vi "RemoteVI Window Rows.vi"(0 "raw":T2(array[cluster]), 1 "labview only?":bool, 2 "skip":u64) -> (4 "rows":T1(array[cluster]))   [LabVIEW 2020, in "RemoteVI.lvlib"]
doc: "The windows RemoteVI Server offers to share, grouped and sorted, from the top-level windows RemoteVI List Top Windows.vi read. Kept: visible, at least 100 x 50 pixels, with a caption, not a tool window (WS_EX_TOOLWINDOW) nor one that cannot be activated (WS_EX_NOACTIVATE), not a shell window (classes Windows.UI.Core.CoreWindow, Windows.Internal.Shell.TabProxyWindow, Progman, LockScreenBackstopFrame); a LabVIEW window (class LVDChild) also when it is owned (LabVIEW's panels are owned by its hidden frame window), other windows only when they are not owned (no dialogs); no LabVIEW window whose caption names a Block Diagram or Project Explorer; not the window skip (the app's own). group 0 = LabVIEW (the development environment, LabVIEW.exe), 1 = a LabVIEW-built application (a LabVIEW window of another program), 2 = other programs; labview only? keeps groups 0 and 1. Sorted by group, program name (case-insensitive) and caption. Pure function, cannot fail. Reference: windowRows() in tools\\lib\\server-app.mjs, vectors tests\\vectors\\server-app.json."
uses:
  RemoteVI.lvlib
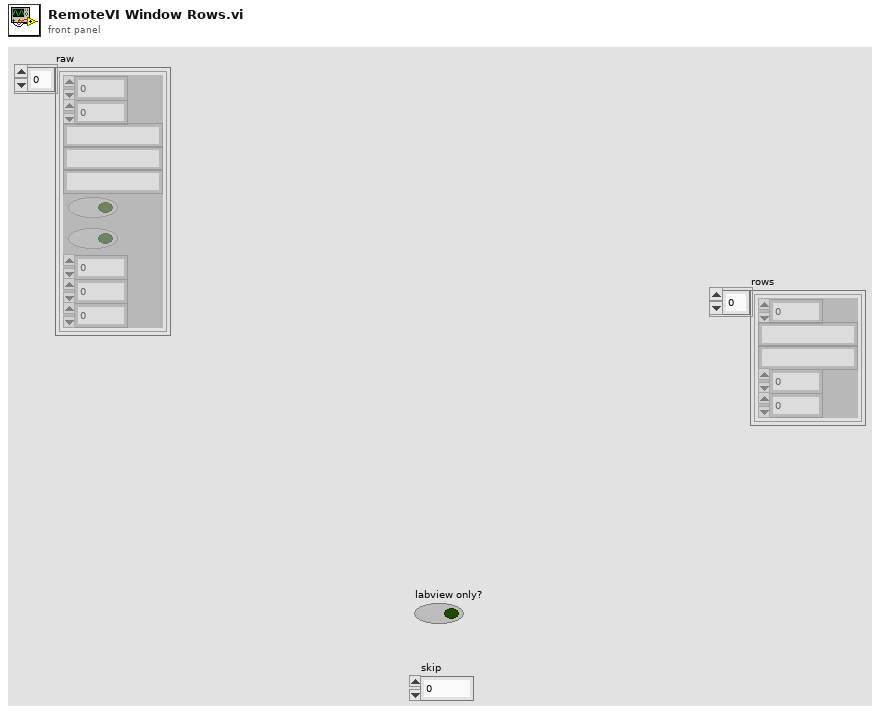
[diagram p1: front panel]
types:
  T1 = cluster{"group":i32, "program":string, "title":string, "pid":u32, "hWnd":u64}[]
  T2 = cluster{"hWnd":u64, "pid":u32, "path":string, "class":string, "title":string, "visible":bool, "owned":bool, "ex style":u32, "w":i32, "h":i32}[]
  T3 = cluster{"group":i32, "program":string, "title":string, "pid":u32, "hWnd":u64}
  T4 = cluster{"group":i32, "key":string, "title":string, "program":string, "pid":u32, "hWnd":u64}
  T5 = cluster{"group":i32, "key":string, "title":string, "program":string, "pid":u32, "hWnd":u64}[]
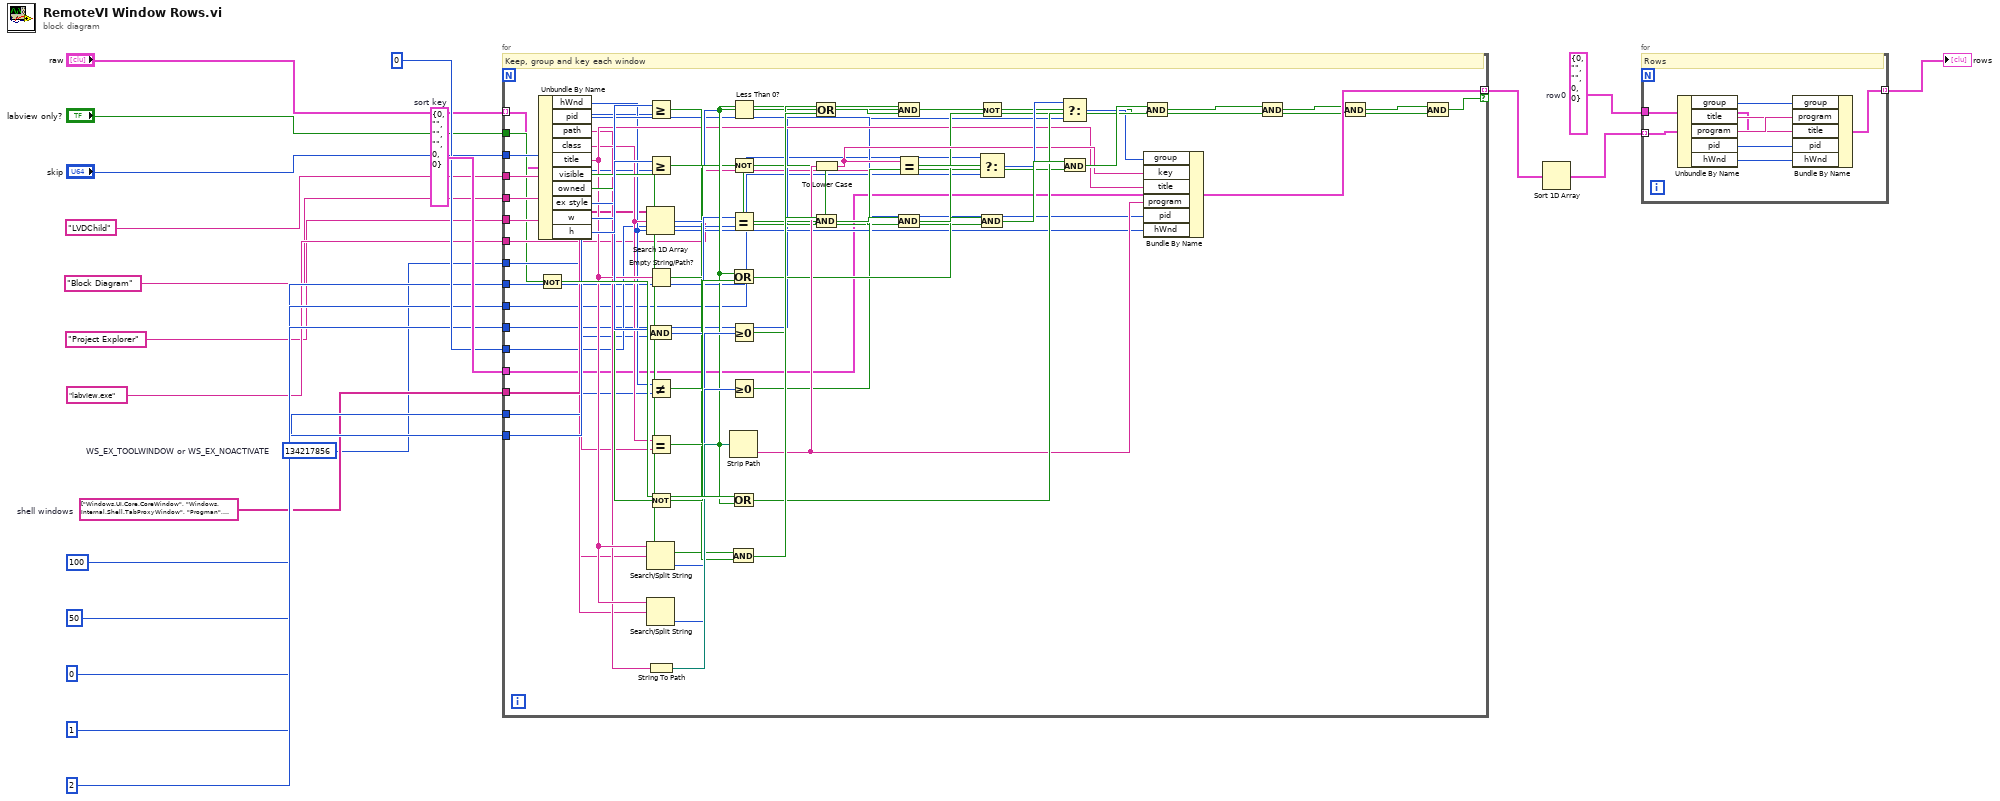
[diagram p0: block diagram]
diagram:
  w19 = T3 {"group"=0, "program"="", "title"="", "pid"=0, "hWnd"=0}  # row0
  w16 = T4 {"group"=0, "key"="", "title"="", "program"="", "pid"=0, "hWnd"=0}  # sort key
  w9 = string[] ["Windows.UI.Core.CoreWindow", "Windows.Internal.Shell.TabProxyWindow", "Progman", "LockScreenBackstopFrame"]  # shell windows
  w8 = u32 134217856  # WS_EX_TOOLWINDOW or WS_EX_NOACTIVATE
  n1 = for {
    tunnel: "raw" -> [w21] mode=indexing
    tunnel: "labview only?" -> [w22]
    tunnel: "skip" -> [w23]
    tunnel: "LVDChild" -> [w24]
    tunnel: "Block Diagram" -> [w25]
    tunnel: "Project Explorer" -> [w26]
    tunnel: "labview.exe" -> [w27]
    tunnel: w8 -> [w28]
    tunnel: 0 -> [w29]
    tunnel: 1 -> [w30]
    tunnel: 2 -> [w31]
    tunnel: u32 0 -> [w32]
    tunnel: w16 -> [w33]
    tunnel: w9 -> [w34]
    tunnel: 100 -> [w35]
    tunnel: 50 -> [w36]
    tunnel: [w83] -> w17 mode=indexing if=w82
    # "Keep, group and key each window"
    n2 = Unbundle By Name(w21) -> ("hWnd"=w37:u64, "pid"=w38:u32, "path"=w39:string, "class"=w40:string, "title"=w41:string, "visible"=w42:bool, "owned"=w43:bool, "ex style"=w44:u32, "w"=w45:i32, "h"=w46:i32)
    n3 = Not(x=w22) -> (.not. x?=w72:bool)
    n4 = Greater Or Equal?(x=w45, y=w35) -> (x >= y?=w47:bool)
    n5 = Greater Or Equal?(x=w46, y=w36) -> (x >= y?=w48:bool)
    n6 = Search 1D Array(1D array=w34, element=w40) -> (index of element=w49:i32)  [unwired: 1 in]
    n7 = Empty String/Path?(string/path=w41) -> (empty?=w51:bool)
    n8 = And(x=w44, y=w28) -> (x .and. y?=w53:u32)
    n9 = Not Equal?(x=w37, y=w23) -> (x != y?=w55:bool)
    n10 = Equal?(x=w40, y=w24) -> (x = y?=w56:bool)
    n11 = Not(x=w43) -> (.not. x?=w57:bool)
    n12 = Search/Split String(string=w41, search string/char (-)=w25) -> (offset of match=w59:i32)  [unwired: 1 in, 2 out]
    n13 = Search/Split String(string=w41, search string/char (-)=w26) -> (offset of match=w60:i32)  [unwired: 1 in, 2 out]
    n14 = String To Path(string=w39) -> (path=w66:path)
    n15 = Less Than 0?(x=w49) -> (x < 0?=w50:bool)
    n16 = Not(x=w51) -> (.not. x?=w52:bool)
    n17 = Equal?(x=w53, y=w32) -> (x = y?=w54:bool)
    n18 = Or(x=w56, y=w57) -> (x .or. y?=w58:bool)
    n19 = Greater Or Equal To 0?(x=w59) -> (x >= 0?=w61:bool)
    n20 = Greater Or Equal To 0?(x=w60) -> (x >= 0?=w62:bool)
    n21 = Strip Path(path=w66) -> (name=w67:string)  [unwired: 1 out]
    n22 = Or(x=w72, y=w56) -> (x .or. y?=w73:bool)
    n23 = And(x=w42, y=w47) -> (x .and. y?=w74:bool)
    n24 = Or(x=w61, y=w62) -> (x .or. y?=w63:bool)
    n25 = To Lower Case(string=w67) -> (all lower case string=w68:string)
    n26 = And(x=w74, y=w48) -> (x .and. y?=w75:bool)
    n27 = And(x=w56, y=w63) -> (x .and. y?=w64:bool)
    n28 = Equal?(x=w68, y=w27) -> (x = y?=w69:bool)
    n29 = And(x=w75, y=w52) -> (x .and. y?=w76:bool)
    n30 = Not(x=w64) -> (.not. x?=w65:bool)
    n31 = Select(t=w29, s=w69, f=w30) -> (s? t:f=w70:i32)
    n32 = And(x=w76, y=w54) -> (x .and. y?=w77:bool)
    n33 = Select(t=w70, s=w56, f=w31) -> (s? t:f=w71:i32)
    n34 = And(x=w77, y=w55) -> (x .and. y?=w78:bool)
    n35 = And(x=w78, y=w58) -> (x .and. y?=w79:bool)
    n36 = Bundle By Name(cluster=w33, "group"=w71, "key"=w68, "title"=w41, "program"=w67, "pid"=w38, "hWnd"=w37) -> (w83:T4)
    n37 = And(x=w79, y=w65) -> (x .and. y?=w80:bool)
    n38 = And(x=w80, y=w73) -> (x .and. y?=w81:bool)
    n39 = And(x=w81, y=w50) -> (x .and. y?=w82:bool)
  }
  n40 = Sort 1D Array(array=w17) -> (sorted array=w18:T5)
  n41 = for {
    tunnel: w19 -> [w85]
    tunnel: w18 -> [w84] mode=indexing
    tunnel: [w91] -> w20 mode=indexing
    # "Rows"
    n42 = Unbundle By Name(w84) -> ("group"=w86:i32, "title"=w87:string, "program"=w88:string, "pid"=w89:u32, "hWnd"=w90:u64)
    n43 = Bundle By Name(cluster=w85, "group"=w86, "program"=w88, "title"=w87, "pid"=w89, "hWnd"=w90) -> (w91:T3)
  }
  "rows" <- w20
